vi "Write Outgoing Bytes.vi"(8 "error in (no error)":errorcluster, 9 "timeout ms (2000)":i32=2000, 10 "Bytes":u8[](array[numeric]) format="%08b", 11 "Connection.TCP":refnum<class "Connection.TCP.lvclass">) -> (0 "error out":errorcluster, 3 "Connection.TCP":refnum<class "Connection.TCP.lvclass">)   [LabVIEW 2013, in "Connection.TCP_GOSPL.lvlib" / "Connection.TCP.lvclass"]
uses:
  Connection.TCP.lvclass
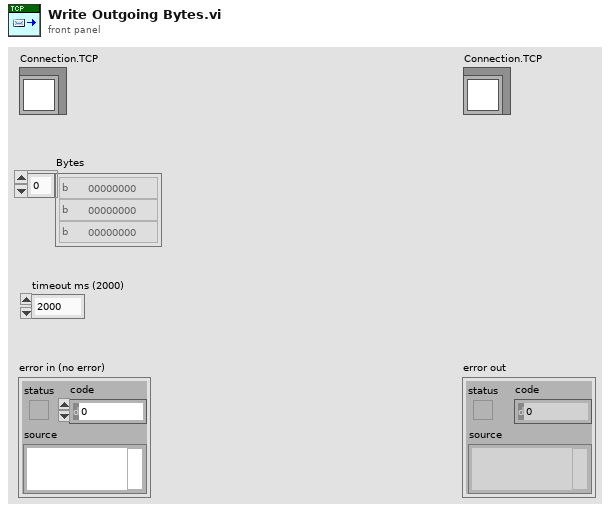
[diagram p1: front panel]
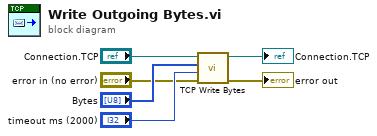
[diagram p0: block diagram]
diagram:
  n1 = call "TCP Write Bytes.vi"("error in (no error)"="error in (no error)", "timeout ms (2000)"="timeout ms (2000)", "Bytes"="Bytes", "Connection.TCP"="Connection.TCP") -> ("error out"=→"error out":errorcluster, "Connection.TCP"=→"Connection.TCP":refnum<class "Connection.TCP.lvclass">)  [unwired: 6 in]
